vi "Variant to String.vi"(8 "error in":errorcluster, 9 "Variant Value":variant) -> (0 "error out":errorcluster, 1 "String Value":string)   [LabVIEW 2020, in "Tag Engine.lvlib"]
doc: "Attempt to represent the input varriant value as a string.\n\nThis VI just calls \"Variant to JSON Text.vi\"\n\nReturned strings are in JSON-compatible value format."
uses:
  Tag Engine.lvlib
  <vilib>/Utility/Data Type/NI_Data Type.lvlib
  <vilib>/JDP Science/JSONtext/JSONtext.lvlib
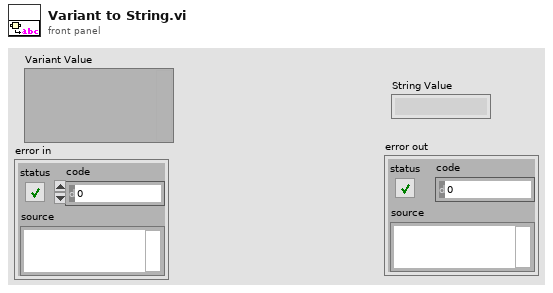
[diagram p1: front panel]
types:
  T1 = typedef "NI_Data Type.lvlib/Data Type.ctl" = enum8{"Invalid Type", "Void", "I8", "I16", "I32", "I64", "U8", "U16", "U32", "U64", "Single Float", "Double Float", "Extended Float", "Single Complex", "Double Complex", "Extended Complex", "Enum U8", "Enum U16", "Enum U32", "Enum U64", "Single Float With Unit", "Double Float With Unit", "Extended Float With Unit", "Single Complex with Unit", "Double Complex with Unit", "Extended Complex with Unit", "Boolean", "String", "Path", "Picture", "Tag", "Array", "Cluster", "Variant", "LV Variant", "Waveform", "Timestamp", "Digital Waveform", "Digital Data", "ExpressData", "Refnum", "External Data", "VI", "Poly VI", "LabVIEW Class Instance", "Fixed Point", "Set Collection", "Map Collection"}
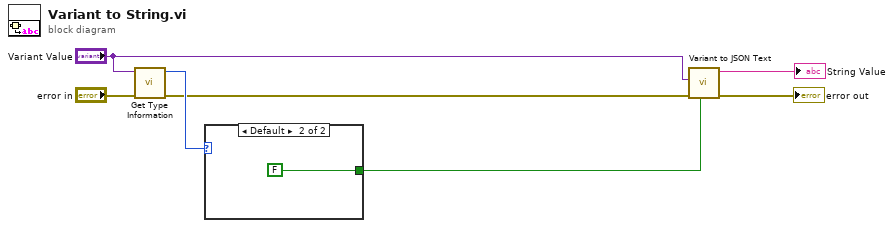
[diagram p0: block diagram]
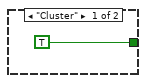
[diagram p2: hidden frame]
diagram:
  n1 = call <vilib>:"Get Type Information.vi"("error in (no error)"="error in", "variant"="Variant Value") -> ("error out"=w1:errorcluster, "type"=w6:T1)  [unwired: 5 in, 3 out]
  n2 = case shown="Default" w6 {
    tunnel: [TRUE ("Pretty Print?") FALSE ("Pretty Print?")] -> w3
    frame "Cluster" {
    }
    frame Default {
    }
  }
  n3 = call <vilib>:"Variant to JSON Text.vi"("Pretty Print?"=w3, "error in (no error)"=w1, "Variant"="Variant Value") -> ("error out"=→"error out":errorcluster, "<JSON>"=→"String Value":string)  [unwired: 6 in, 1 out]
